vi "test Parse System Definition to Create Tx Execution Units.vi"(8 "error in":errorcluster, 11 "TestCase in":refnum<class "Engine.lvclass">) -> (0 "error out":errorcluster, 3 "TestCase out":refnum<class "Engine.lvclass">)   [LabVIEW 2020, in "Engine.lvclass"]
uses:
  Engine.lvclass
  Engine.lvclass/Engine.ctl
  C:/Program Files/National Instruments/LabVIEW 2026/vi.lib/addons/_JKI Toolkits/VI Tester/TestCase.llb/TestCase.lvclass
  C:/git/fmussi_niveristand-aim-arinc429-custom-device/Source/Custom Device Support/Tests/Unit/Execution/Engine/Engine.lvclass
  <vilib>/addons/_JKI Toolkits/VI Tester/TestCase.llb/TestCase.lvclass
  <vilib>/NI/VeriStand Custom Device Testing Tools/VeriStandTestUtilities/VeriStandTestUtilities.lvlib
  <userlib>/_OpenG.lib/appcontrol/appcontrol.llb/openg_application_control.lvlib
  Scripting/AIM/AIM ARINC 429 Scripting.lvlib
  Engine/Implementation/Execution Unit Factory/Execution Unit Factory.lvclass
  Engine/Implementation/Tx Acyclic Labels Execution Unit/Tx Acyclic Labels Execution Unit.lvclass
  Engine/Implementation/Tx Scheduled Labels Execution Unit/Tx Scheduled Labels Execution Unit.lvclass
  <vilib>/NI VeriStand/Custom Device API/Data Reference.ctl
  <vilib>/NI VeriStand/Custom Device API/Custom Device API.lvlib
  <vilib>/NI VeriStand/Custom Device API/Custom Device Item Ref.ctl
  Shared/Transfer Type.ctl
  <vilib>/NI/NI VeriStand Encoding and Decoding/Encoding.ctl
  <vilib>/NI/NI VeriStand Encoding and Decoding/Encoding and Decoding.lvlib
  Shared/Parameter Definition.ctl
  Shared/RT Parameters.ctl
  Shared/Label.ctl
  Shared/RT Label Settings.ctl
  Shared/RT Hardware Channel Settings.ctl
  Shared/Transfer Speed.ctl
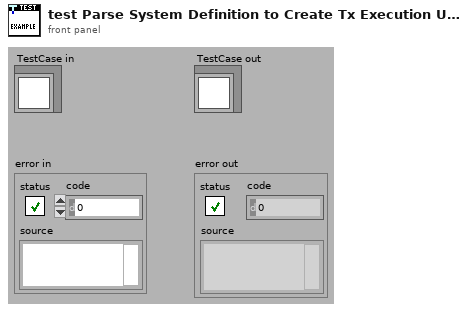
[diagram p1: front panel]
types:
  T1 = typedef "RT Hardware Channel Settings.ctl" = cluster{"channel #":u16, "channel handle":u64, "labels settings for RT":T2[], "speed":T10}
  T2 = typedef "RT Label Settings.ctl" = cluster{"Name":string, "xmlName":string, "label":T3, "transfer period":u32, "SDI_Enabled":bool, "SDI":u8, "parameter driver data":T4, "transfer type":T8, "has timestamp?":bool, "Label Disable/Trigger Channel Reference":T7, "Message Handle":u64, "Initialized?":bool, "Word Initial Raw Value":u32, "Label Timestamp Channel Data Reference":T9, "disabled":bool, "modified":bool}
  T3 = typedef "Label.ctl" = u8
  T4 = typedef "RT Parameters.ctl" = cluster{"parameter definitions":T5[], "Tx parameter refs":T7[]}
  T5 = typedef "Parameter Definition.ctl" = cluster{"start index":i32, "size":i32, "encoding":T6, "signed":bool, "scale multiplier":dbl, "scale offset":dbl, "default value":dbl}
  T6 = typedef "Encoding and Decoding.lvlib/Encoding.ctl" = enum16{"BNR", "BCD", "Discrete"}
  T7 = typedef "Custom Device API.lvlib/Custom Device Item Ref.ctl" = u64
  T8 = typedef "Transfer Type.ctl" = enum16{"Scheduled", "Acyclic", "Block", "Strobe"}
  T9 = typedef "Custom Device API.lvlib/Data Reference.ctl" = i32
  T10 = typedef "Transfer Speed.ctl" = enum16{"LO (12.5 kb/s)", "HI (100 kb/s)"}
  T11 = typedef "AIM ARINC 429 Engine.lvlib/Interfaces.lvlib/Execution Unit Information.ctl" = cluster{"Execution Unit":refnum<class "Execution Unit.lvclass">, "Incoming Channels":T7[], "Outgoing Channels":T7[], "ReadWrite Channels":T7[]}
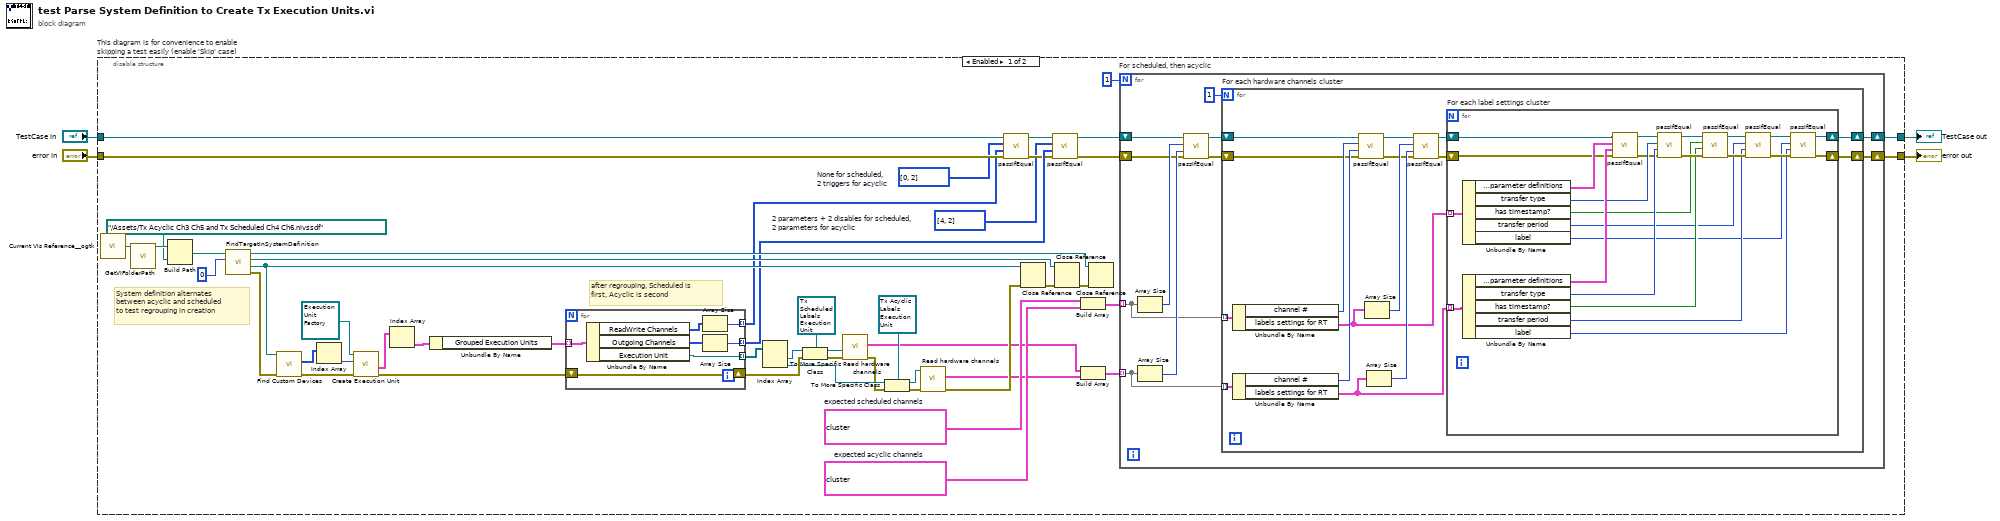
[diagram p0: block diagram]
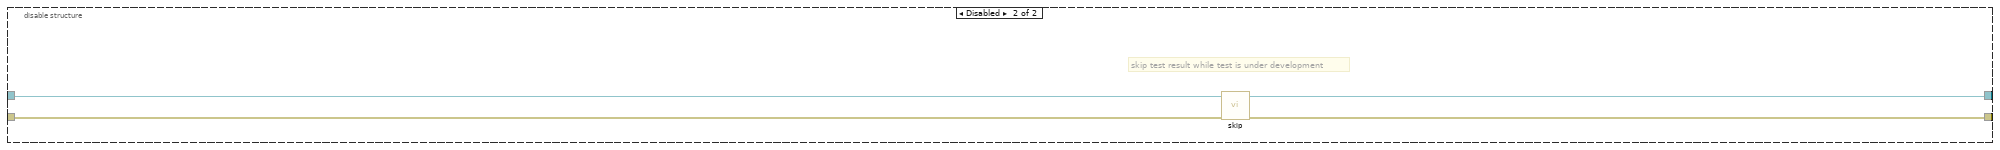
[diagram p2: hidden frame]
diagram:
  n1 = disable-structure "This diagram is for convenience to enable skipping a test easily (enable 'Skip' case)" shown="Enabled" {
    disable-tunnel: "TestCase in" -> [w54 w116]
    disable-tunnel: [w42 w114] -> w1
    disable-tunnel: [w41 w115] -> w3
    disable-tunnel: "error in" -> [w53 w113]
    frame Enabled {
      w12 = T1[] [{"channel #"=3, "channel handle"=0, "labels settings for RT"=[{"Name"="label 81", "xmlName"="", "label"=81, "transfer period"=10, "SDI_Enabled"=FALSE, "SDI"=0, "parameter driver data"={"parameter definitions"=[{"start index"=10, "size"=19, "encoding"=enum."BNR", "signed"=TRUE, "scale multiplier"=1.0, "scale offset"=0.0, "default value"=0.0}], "Tx parameter refs"=[35]}, "transfer type"=enum."Acyclic", "has timestamp?"=FALSE, "Label Disable/Trigger Channel Reference"=36, "Message Handle"=0, "Initialized?"=TRUE, "Word Initial Raw Value"=0, "Label Timestamp Channel Data Reference"=0, "disabled"=FALSE, "modified"=FALSE}], "speed"=enum."HI (100 kb/s)"}, {"channel #"=5, "channel handle"=0, "labels settings for RT"=[{"Name"="label 83", "xmlName"="", "label"=83, "transfer period"=30, "SDI_Enabled"=FALSE, "SDI"=0, "parameter driver data"={"parameter definitions"=[{"start index"=10, "size"=19, "encoding"=enum."BNR", "signed"=FALSE, "scale multiplier"=1.0, "scale offset"=0.0, "default value"=0.0}], "Tx parameter refs"=[45]}, "transfer type"=enum."Acyclic", "has timestamp?"=FALSE, "Label Disable/Trigger Channel Reference"=46, "Message Handle"=0, "Initialized?"=TRUE, "Word Initial Raw Value"=0, "Label Timestamp Channel Data Reference"=0, "disabled"=FALSE, "modified"=FALSE}], "speed"=enum."HI (100 kb/s)"}]  # expected acyclic channels
      w14 = T1[] [{"channel #"=4, "channel handle"=0, "labels settings for RT"=[{"Name"="label 82", "xmlName"="", "label"=82, "transfer period"=20, "SDI_Enabled"=FALSE, "SDI"=0, "parameter driver data"={"parameter definitions"=[{"start index"=10, "size"=19, "encoding"=enum."BNR", "signed"=TRUE, "scale multiplier"=1.0, "scale offset"=0.0, "default value"=0.0}], "Tx parameter refs"=[40]}, "transfer type"=enum."Scheduled", "has timestamp?"=FALSE, "Label Disable/Trigger Channel Reference"=41, "Message Handle"=0, "Initialized?"=TRUE, "Word Initial Raw Value"=0, "Label Timestamp Channel Data Reference"=0, "disabled"=FALSE, "modified"=FALSE}], "speed"=enum."HI (100 kb/s)"}, {"channel #"=6, "channel handle"=0, "labels settings for RT"=[{"Name"="label 84", "xmlName"="", "label"=84, "transfer period"=40, "SDI_Enabled"=FALSE, "SDI"=0, "parameter driver data"={"parameter definitions"=[{"start index"=10, "size"=19, "encoding"=enum."BNR", "signed"=FALSE, "scale multiplier"=1.0, "scale offset"=0.0, "default value"=0.0}], "Tx parameter refs"=[50]}, "transfer type"=enum."Scheduled", "has timestamp?"=FALSE, "Label Disable/Trigger Channel Reference"=51, "Message Handle"=0, "Initialized?"=TRUE, "Word Initial Raw Value"=0, "Label Timestamp Channel Data Reference"=0, "disabled"=FALSE, "modified"=FALSE}], "speed"=enum."HI (100 kb/s)"}]  # expected scheduled channels
      w16 = i32[] [4, 2]  # 2 parameters + 2 disables for scheduled, 2 parameters for acyclic
      w17 = i32[] [0, 2]  # None for scheduled, 2 triggers for acyclic
      # "System definition alternates\nbetween acyclic and scheduled\nto test regrouping in creation"
      # "after regrouping, Scheduled is \nfirst, Acyclic is second"
      n2 = call <userlib>:"Current VIs Reference__ogtk.vi"() -> ("Current VI's reference"=w44:refnum<vi>)  [unwired: 5 in]
      n3 = call <vilib>:"GetVIFolderPath.vi"("VI Reference in"=w44) -> ("VI Folder Path out"=w45:path)  [unwired: 9 in, 1 out]
      n4 = Build Path(base path=w45, name or relative path=path "../Assets/Tx Acyclic Ch3 Ch5 and Tx Scheduled Ch4 Ch6.nivssdf" ("system definition path")) -> (appended path=w43:path)
      n5 = call <vilib>:"FindTargetInSystemDefinition.vi"("target index"=0 ("index"), "system definition path"=w43) -> ("error out"=w46:errorcluster, "Target"=w49:refnum<k24>, "Root"=w48:refnum<k24>, "System Definition"=w47:refnum<k24>)  [unwired: 6 in]
      n6 = call "Find Custom Devices.vi"("error in"=w46, "target"=w49) -> ("error out"=w37:errorcluster, "AIM ARINC 429 custom devices"=w39:T7[])  [unwired: 7 in, 1 out]
      n7 = Index Array(array=w39) -> (element=w38:T7)  [unwired: 1 in]
      n8 = call-dynamic "Create Execution Unit.vi"("error in"=w37, "Item Ref"=w38, "Execution Unit Factory Implementation in"=refnum<class "Execution Unit Factory.lvclass"> refnum ("Communication Bus Template Interfaces:Implementation.lvlib:Execution Unit Factory.lvclass")) -> ("error out"=w35:errorcluster, "Asynchronous Execution Units"=w7:cluster{"Grouped Execution Units":T11[]}[])  [unwired: 5 in, 2 out]
      n9 = Index Array(array=w7) -> (element=w6:cluster{"Grouped Execution Units":T11[]})  [unwired: 1 in]
      n10 = Unbundle By Name(w6) -> ("Grouped Execution Units"=w5:T11[])
      n11 = for {
        shift-right: [w112] -> w28
        shift-left: w35 -> [w112]
        tunnel: [w111] -> w29 mode=indexing
        tunnel: [w109] -> w34 mode=indexing
        tunnel: [w110] -> w15 mode=indexing
        tunnel: w5 -> [w106] mode=indexing
        n12 = Unbundle By Name(w106) -> ("ReadWrite Channels"=w107:T7[], "Outgoing Channels"=w108:T7[], "Execution Unit"=w111:refnum<class "Execution Unit.lvclass">)
        n13 = Array Size(array=w107) -> (size(s)=w110:i32)
        n14 = Array Size(array=w108) -> (size(s)=w109:i32)
      }
      n15 = Index Array(array=w29) -> (element #1=w26:refnum<class "Execution Unit.lvclass">, element #2=w25:refnum<class "Execution Unit.lvclass">)  [unwired: 2 in]
      n16 = To More Specific Class(target class=refnum<class "Tx Scheduled Labels Execution Unit.lvclass"> refnum ("Communication Bus Template Interfaces:Implementation.lvlib:Tx Scheduled Labels Execution Unit.lvclass"), reference=w26, error in=w28) -> (specific class reference=w23:refnum<class "Tx Scheduled Labels Execution Unit.lvclass">, error out=w22:errorcluster)
      n17 = call "Read hardware channels.vi"("error in (no error)"=w22, "Tx Scheduled Labels Execution Unit in"=w23) -> ("error out"=w21:errorcluster, "hardware channels"=w10:T1[])  [unwired: 7 in, 1 out]
      n18 = To More Specific Class(target class=refnum<class "Tx Acyclic Labels Execution Unit.lvclass"> refnum ("Communication Bus Template Interfaces:Implementation.lvlib:Tx Acyclic Labels Execution Unit.lvclass"), reference=w25, error in=w21) -> (specific class reference=w19:refnum<class "Tx Acyclic Labels Execution Unit.lvclass">, error out=w20:errorcluster)
      n19 = call "Read hardware channels.vi"("error in (no error)"=w20, "Tx Acyclic Labels Execution Unit in"=w19) -> ("error out"=w18:errorcluster, "hardware channels"=w9:T1[])  [unwired: 7 in, 1 out]
      n20 = call-dynamic "passIfEqual.vi"("error in (no error)"=w53, "y"=w15, "x"=w17, "TestCase in"=w54) -> ("error out"=w33:errorcluster, "TestCase out"=w31:refnum<class "Engine.lvclass">)  [unwired: 6 in]
      n21 = Close Reference(reference=w49, error in (no error)=w18) -> (error out=w51:errorcluster)
      n22 = call-dynamic "passIfEqual.vi"("error in (no error)"=w33, "y"=w34, "x"=w16, "TestCase in"=w31) -> ("error out"=w32:errorcluster, "TestCase out"=w30:refnum<class "Engine.lvclass">)  [unwired: 6 in]
      n23 = Close Reference(reference=w48, error in (no error)=w51) -> (error out=w50:errorcluster)
      n24 = Build Array(w14, w12) -> (w13:T1[][])
      n25 = Build Array(w10, w9) -> (w11:T1[][])
      n26 = Close Reference(reference=w47, error in (no error)=w50) -> ()  [unwired: 1 out]
      n27 = for "For scheduled, then acyclic" {
        N: 1 -> [_]
        tunnel: w11 -> [w57] mode=indexing
        tunnel: w13 -> [w56] mode=indexing
        shift-right: [w62] -> w41
        shift-left: w32 -> [w61]
        shift-right: [w63] -> w42
        shift-left: w30 -> [w60]
        n28 = Array Size(array=w56) -> (size(s)=w65:i32)
        n29 = Array Size(array=w57) -> (size(s)=w64:i32)
        n30 = call-dynamic "passIfEqual.vi"("error in (no error)"=w61, "y"=w64, "x"=w65, "TestCase in"=w60) -> ("error out"=w58:errorcluster, "TestCase out"=w59:refnum<class "Engine.lvclass">)  [unwired: 6 in]
        n31 = for "For each hardware channels cluster" {
          N: 1 -> [_]
          tunnel: w56 -> [w81] mode=indexing
          shift-right: [w67] -> w63
          shift-left: w59 -> [w78]
          shift-right: [w66] -> w62
          shift-left: w58 -> [w77]
          tunnel: w57 -> [w72] mode=indexing
          n32 = Unbundle By Name(w81) -> ("channel #"=w80:u16, "labels settings for RT"=w68:T2[])
          n33 = Unbundle By Name(w72) -> ("channel #"=w79:u16, "labels settings for RT"=w69:T2[])
          n34 = call-dynamic "passIfEqual.vi"("error in (no error)"=w77, "y"=w79, "x"=w80, "TestCase in"=w78) -> ("error out"=w73:errorcluster, "TestCase out"=w74:refnum<class "Engine.lvclass">)  [unwired: 6 in]
          n35 = Array Size(array=w68) -> (size(s)=w76:i32)
          n36 = Array Size(array=w69) -> (size(s)=w75:i32)
          n37 = call-dynamic "passIfEqual.vi"("error in (no error)"=w73, "y"=w75, "x"=w76, "TestCase in"=w74) -> ("error out"=w71:errorcluster, "TestCase out"=w70:refnum<class "Engine.lvclass">)  [unwired: 6 in]
          n38 = for "For each label settings cluster" {
            tunnel: w68 -> [w105] mode=indexing
            tunnel: w69 -> [w96] mode=indexing
            shift-right: [w85] -> w67
            shift-left: w70 -> [w98]
            shift-right: [w84] -> w66
            shift-left: w71 -> [w97]
            n39 = Unbundle By Name(w105) -> ("parameter driver data.parameter definitions"=w104:T5[], "transfer type"=w102:T8, "has timestamp?"=w91:bool, "transfer period"=w89:u32, "label"=w82:T3)
            n40 = Unbundle By Name(w96) -> ("parameter driver data.parameter definitions"=w103:T5[], "transfer type"=w101:T8, "has timestamp?"=w90:bool, "transfer period"=w88:u32, "label"=w83:T3)
            n41 = call-dynamic "passIfEqual.vi"("error in (no error)"=w97, "y"=w103, "x"=w104, "TestCase in"=w98) -> ("error out"=w99:errorcluster, "TestCase out"=w100:refnum<class "Engine.lvclass">)  [unwired: 6 in]
            n42 = call-dynamic "passIfEqual.vi"("error in (no error)"=w99, "y"=w101, "x"=w102, "TestCase in"=w100) -> ("error out"=w95:errorcluster, "TestCase out"=w94:refnum<class "Engine.lvclass">)  [unwired: 6 in]
            n43 = call-dynamic "passIfEqual.vi"("error in (no error)"=w95, "y"=w90, "x"=w91, "TestCase in"=w94) -> ("error out"=w93:errorcluster, "TestCase out"=w92:refnum<class "Engine.lvclass">)  [unwired: 6 in]
            n44 = call-dynamic "passIfEqual.vi"("error in (no error)"=w93, "y"=w88, "x"=w89, "TestCase in"=w92) -> ("error out"=w87:errorcluster, "TestCase out"=w86:refnum<class "Engine.lvclass">)  [unwired: 6 in]
            n45 = call-dynamic "passIfEqual.vi"("error in (no error)"=w87, "y"=w83, "x"=w82, "TestCase in"=w86) -> ("error out"=w84:errorcluster, "TestCase out"=w85:refnum<class "Engine.lvclass">)  [unwired: 6 in]
          }
        }
      }
    }
    frame Disabled {
      # "skip test result while test is under development"
      n46 = call <vilib>:"skip.vi"("error in (no error)"=w113, "TestCase in"=w116) -> ("error out"=w115:errorcluster, "TestCase out"=w114:refnum<class "Engine.lvclass">)  [unwired: 8 in]
    }
  }
  "error out" <- w3
  "TestCase out" <- w1
